vi "RT Main2.vi"   [LabVIEW 2025]
uses:
  <vilib>/NI_Real-Time Target Support.lvlib
  <resource>/objmgr/nisysapi.rc
  <vilib>/nisyscfg/nisyscfg.lvlib
types:
  T1 = typedef "NI_Real-Time Target Support.lvlib/RT CPU Load.ctl" = cluster{"Total (%)":dbl, "Time Critical (%)":dbl, "Timed Structures (%)":dbl, "High (%)":dbl, "Above Normal (%)":dbl, "Normal (%)":dbl, "Background (%)":dbl, "Idle (%)":dbl, "ISR (%)":dbl}
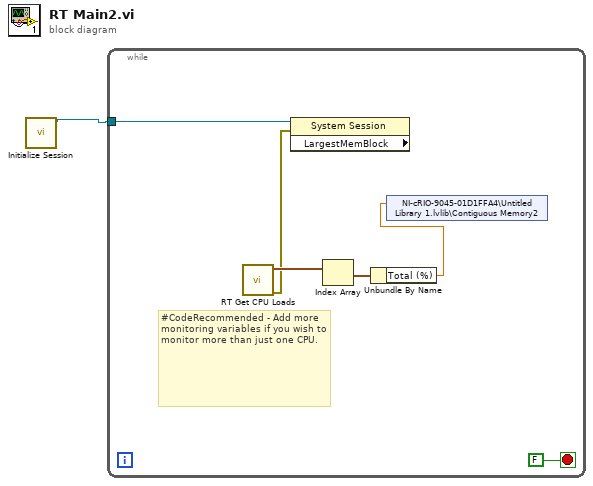
[diagram p0: block diagram]
diagram:
  n1 = call <vilib>:"Initialize Session.vi"() -> ("Session out"=w1:refnum<k21>)  [unwired: 10 in, 1 out]
  n2 = while {
    tunnel: w1 -> [w4]
    stop <- FALSE stop-if-true
    # "#CodeRecommended - Add more monitoring variables if you wish to monitor more than just one CPU."
    n3 = call <vilib>:"RT Get CPU Loads.vi"() -> ("error out"=w5:errorcluster, "CPU loads"=w7:T1[])  [unwired: 10 in]
    n4 = property class="System Session" props=["LargestMemBlock"](reference=w4, error in=w5) -> ()  [unwired: 3 out]
    n5 = Index Array(array=w7) -> (element=w6:T1)  [unwired: 1 in]
    n6 = Unbundle By Name(w6) -> ("Total (%)"=w2:dbl)
    n7 = shared-variable "NI-cRIO-9045-01D1FFA4\\Untitled Library 1.lvlib\\Contiguous Memory2"(w2) -> ()  [unwired: 1 in, 1 out]
  }
